vi "GpuMat Reshape.vi"(8 "error in (no error)":errorcluster, 9 "rows":i32, 10 "cn":i32, 11 "GpuMat in":refnum<class "GpuMat.lvclass">) -> (0 "error out":errorcluster, 2 "Dst out":refnum<class "GpuMat.lvclass">, 3 "GpuMat out":refnum<class "GpuMat.lvclass">)   [LabVIEW 2020, in "OpenLvVision_OpenCv.lvlib" / "Cuda.lvlib" / "GpuMat.lvclass"]
doc: "Creates alternative GpuMat header for the same data, with different number of channels and/or different number of rows"
uses:
  GpuMat.lvclass
  C:/Users/lukas/Documents/OpenLvVision_OpenCv/SourceCode/LabView/OpenLvVision_OpenCv/_LvHelpers/EdvrObject/EdvrObject.lvclass
  _LvHelpers/EdvrObject/EdvrObject.lvclass/EdvrObject.ctl
  _LvHelpers/EdvrObject/TypeDef/Edvr.ctl
  OpenLvVision_OpenCv.lvlib
  <vilib>/Utility/error.llb/Error Cluster From Error Code.vi
  <vilib>/ErrorRing/Error Ring.xnode
  _LvHelpers/EdvrObject/EdvrObject.lvclass
  Dlls/OlvOpenCvWrapper.dll
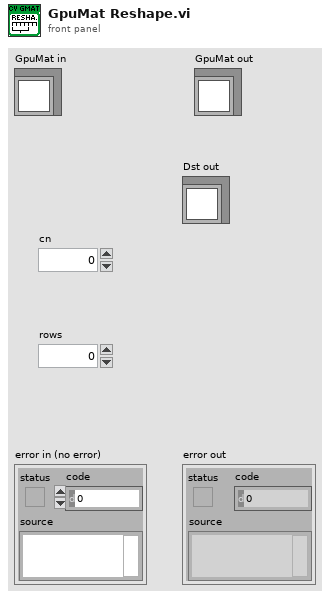
[diagram p1: front panel]
types:
  T1 = typedef "OpenLvVision_OpenCv.lvlib/EdvrObject.lvclass/Edvr.ctl" = refnum<data-value>
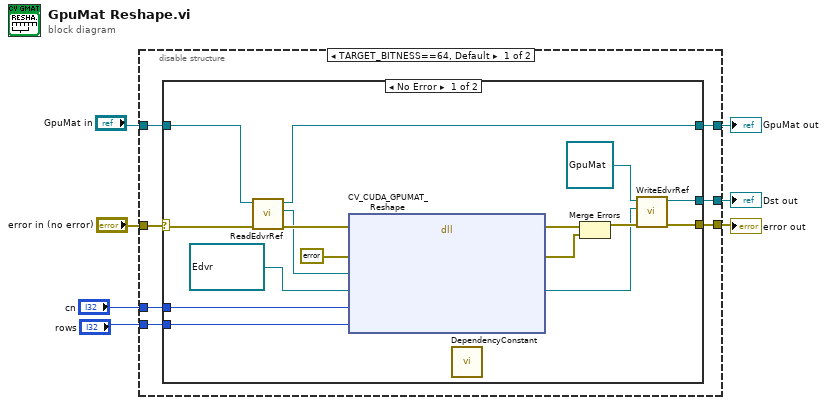
[diagram p0: block diagram]
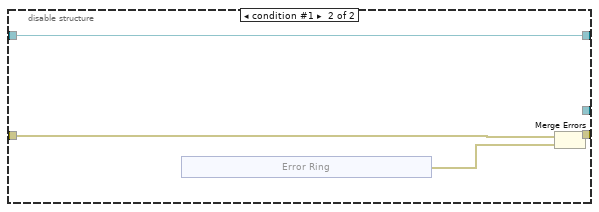
[diagram p3: hidden frame]
diagram:
  n1 = disable-structure shown="TARGET_BITNESS==64, Default" {
    disable-tunnel: "error in (no error)" -> [w14 w35]
    disable-tunnel: [w13 w36] -> w7
    disable-tunnel: "GpuMat in" -> [w12 w33]
    disable-tunnel: [w11 w33] -> w4
    disable-tunnel: "rows" -> [w10 _]
    disable-tunnel: "cn" -> [w9 _]
    disable-tunnel: [w8 _] -> w1
    frame condition #0 (active) {
      n2 = case shown="No Error" w14 {
        selector: w14 -> [w23 w32]
        tunnel: [w18 w32] -> w13
        tunnel: w12 -> [w26 w31]
        tunnel: [w24 w31] -> w11
        tunnel: w10 -> [w22 _]
        tunnel: w9 -> [w21 _]
        tunnel: [w16 _] -> w8
        frame No Error {
          n3 = call "ReadEdvrRef.vi"("error in (no error)"=w23, "EdvrObject in"=w26) -> ("error out"=w27:errorcluster, "Edvr"=w25:T1, "EdvrObject out"=w24:refnum<class "GpuMat.lvclass">)  [unwired: 7 in]
          n4 = dll-call lib="C:/Users/lukas/Documents/OpenLvVision_OpenCv/SourceCode/LabView/OpenLvVision_OpenCv/Dlls/OlvOpenCvWrapper.dll" fn="CV_CUDA_GPUMAT_Reshape"(error in=w27, "Error"=errorcluster {"status"=FALSE, "code"=0, "source"=""} ("error out"), "SrcEdvrRef"=w25, "DstEdvrRef"=T1 refnum ("Edvr"), "cn"=w21, "rows"=w22) -> (error out=w30:errorcluster, "Error"=w29:errorcluster, "DstEdvrRef"=w17:T1)  [unwired: 6 in, 1 out]
          n5 = call "DependencyConstant.vi"() -> ()  [unwired: 12 in]
          n6 = Merge Errors(w30, w29) -> (w19:errorcluster)
          n7 = call "WriteEdvrRef.vi"("error in (no error)"=w19, "Edvr"=w17, "EdvrObject in"=refnum<class "GpuMat.lvclass"> refnum ("GpuMat out")) -> ("error out"=w18:errorcluster, "EdvrObject out"=w16:refnum<class "GpuMat.lvclass">)  [unwired: 7 in]
        }
        frame Error {
        }
      }
    }
    frame condition #1 {
      n8 = xnode "Error Ring"() -> ("error out"=w34:errorcluster)
      n9 = Merge Errors(w35, w34) -> (w36:errorcluster)
    }
  }
  "error out" <- w7
  "GpuMat out" <- w4
  "Dst out" <- w1
